vi "Update Engine.vi"(8 "error in (no error)":errorcluster, 10 "tdms ref":refnum<k34>, 11 "Abstract Engine":refnum<class "Abstract Engine.lvclass">) -> (0 "error out":errorcluster, 3 "Abstract Engine out":refnum<class "Abstract Engine.lvclass">)   [LabVIEW 2025, in "Abstract Engine.lvlib" / "Abstract Engine.lvclass"]
uses:
  Abstract Engine.lvclass
  Abstract Instrument/Abstract Instrument.lvclass
  Abstract Engine.lvclass/Abstract Engine.ctl
  Read Engine Cluster.vi
  Users/Public/Documents/Sandia National Labs/TSS Plugin/CEF.lvlibp/Node/ReadChildren.vi
  Users/Public/Documents/Sandia National Labs/TSS Plugin/CEF.lvlibp/Node/CEF_Node.lvclass
  Users/Public/Documents/Sandia National Labs/TSS Plugin/CEF.lvlibp
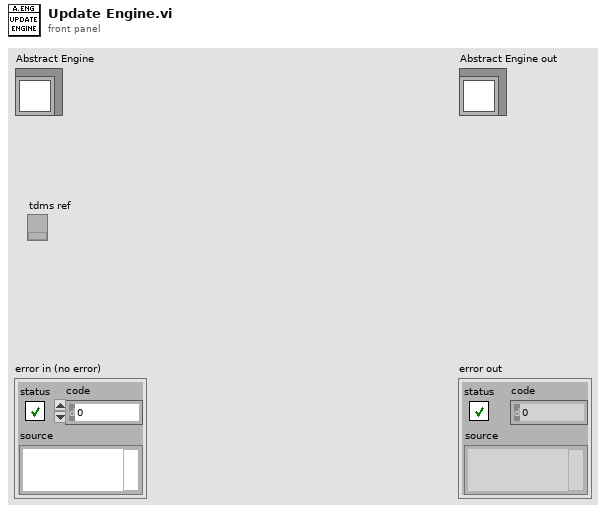
[diagram p1: front panel]
types:
  T1 = typedef "Abstract Engine.lvlib/Abstract Engine.lvclass/Engine Cluster.ctl" = cluster{"IP Address":string, "Type":string, "Initialized":bool, "InstrumentMap":map{string, cluster{"Initialized":bool, "Channels":T2[]}}}
  T2 = typedef "Abstract Engine.lvlib/Abstract Instrument.lvclass/Channel.ctl" = cluster{"Alias":string, "DataType":T3, "Unit":enum16{"---", "V", "A", "Ohm", "Hz", "uF", "degC", "deg"}, "Upper limit":dbl, "Lower limit":dbl, "Measurement":variant}
  T3 = typedef "Abstract Engine.lvlib/Abstract Instrument.lvclass/Data Type.ctl" = string
  T4 = map{string, cluster{"Initialized":bool, "Channels":T2[]}}
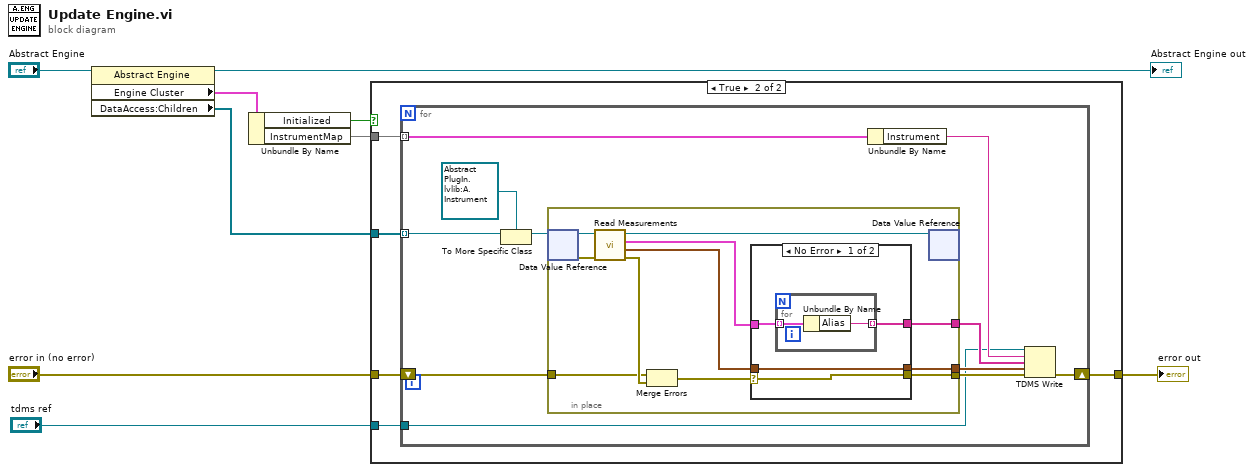
[diagram p0: block diagram]
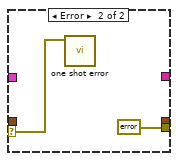
[diagram p3: hidden frame]
diagram:
  n1 = property class="Abstract Engine"(reference="Abstract Engine") -> (reference out=→"Abstract Engine out":refnum<class "Abstract Engine.lvclass">, "Engine Cluster"=w6:T1, "DataAccess:Children"=w8:refnum<data-value>[])  [unwired: 1 in, 1 out]
  n2 = Unbundle By Name(w6) -> ("Initialized"=w7:bool, "InstrumentMap"=w2:T4)
  n3 = case shown="True" w7 {
    tunnel: w8 -> [_ w15]
    tunnel: "error in (no error)" -> [w10 w14]
    tunnel: [w10 w13] -> w4
    tunnel: "tdms ref" -> [_ w12]
    tunnel: w2 -> [_ w11]
    frame False {
    }
    frame True {
      n4 = for {
        tunnel: w15 -> [w26] mode=indexing
        shift-right: [w22] -> w13
        shift-left: w14 -> [w24]
        tunnel: w12 -> [w17]
        tunnel: w11 -> [w20] mode=indexing
        n5 = To More Specific Class(target class=refnum<data-value> refnum ("data value reference"), reference=w26) -> (specific class reference=w25:refnum<data-value>)  [unwired: 1 in, 1 out]
        n6 = in-place {
          in-place-border: w24 -> [w33]
          in-place-border: [w27] -> w23
          in-place-border: [w31] -> w21
          in-place-border: [w28] -> w18
          n7 = in-place-dvr #1(w25) -> (w37:refnum<class "Abstract Instrument.lvclass">, w35:errorcluster)
          n8 = call-dynamic "Read Measurements.vi"("error in (no error)"=w35, "Abs Instrument in"=w37) -> ("error out"=w34:errorcluster, "Waveforms"=w29:waveform(dbl)[], "Measurements"=w32:T2[], "Abs Instrument out"=w36:refnum<class "Abstract Instrument.lvclass">)  [unwired: 6 in]
          n9 = Merge Errors(w33, w34) -> (w30:errorcluster)
          n10 = case shown="No Error" w30 {
            selector: w30 -> [w38 w45]
            tunnel: w32 -> [w41 _]
            tunnel: [w40 _] -> w31
            tunnel: w29 -> [w39 _]
            tunnel: [w39 _] -> w28
            tunnel: [w38 errorcluster {"status"=FALSE, "code"=0, "source"=""} ("error IO")] -> w27
            frame No Error {
              n11 = for {
                tunnel: w41 -> [w43] mode=indexing
                tunnel: [w42] -> w40 mode=indexing
                n12 = Unbundle By Name(w43) -> ("Alias"=w42:string)
              }
            }
            frame Error {
              n13 = call "one shot error.vi"("error in"=w45) -> ()  [unwired: 11 in]
            }
          }
          n14 = in-place-dvr #1(w36) -> ()  [unwired: 2 out]
        }
        n15 = Unbundle By Name(w20) -> ("Instrument"=w19:string)
        n16 = TDMS Write(0:w17, 5:w19, 7:w21, 9:w18, 11:w23) -> (15:w22:errorcluster)  [unwired: 1 in, 3 out]
      }
    }
  }
  "error out" <- w4
